vi "GetPanelUI.vi"(8 "error in (no error)":errorcluster, 11 "object in":refnum<class "DIO-Configuration.lvclass">) -> (0 "error out":errorcluster, 2 "VI Refnum":refnum<vi>, 3 "object out":refnum<class "DIO-Configuration.lvclass">)   [LabVIEW 2021, in "DIO-Channel.lvlib" / "DIO-Configuration.lvclass"]
uses:
  DIO-Configuration.lvclass
  DIO-Configuration.lvclass/DIO-Configuration.ctl
  DIO-Panel.vi
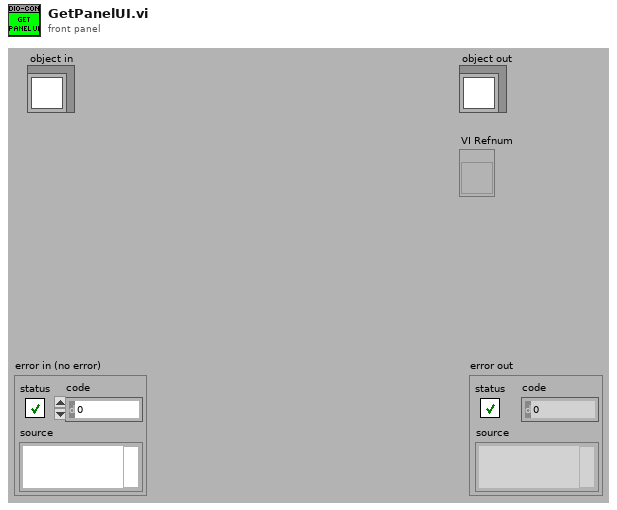
[diagram p1: front panel]
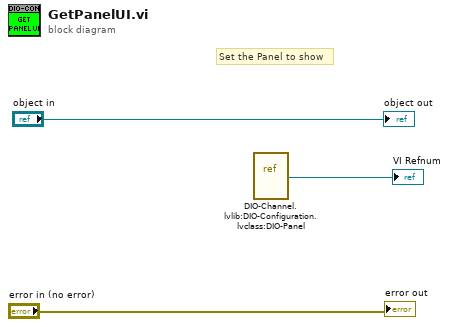
[diagram p0: block diagram]
diagram:
  # "Set the Panel to show"
  n1 = vi-ref "DIO-Channel.lvlib:DIO-Configuration.lvclass:DIO-Panel.vi"() -> (→"VI Refnum":refnum<vi>)
  "error out" <- "error in (no error)"
  "object out" <- "object in"
